vi "VIH Utility - FILE - Save File Dialog.vi"(4 "pattern label":string, 5 "button label":string, 6 "pattern":string, 7 "prompt":string, 8 "error in":errorcluster, 9 "default name":string, 11 "start path":path) -> (0 "error out":errorcluster, 2 "exists":bool, 3 "File path":path)   [LabVIEW 2014]
doc: "::: VI Helpeks :::\nCopyright (c) 2000-2026 Konstantin Shifershteyn. All rights reserved."
panel:
  # "VI Helpeks\nCopyright (c) 2012-2026 Konstantin Shifershteyn"
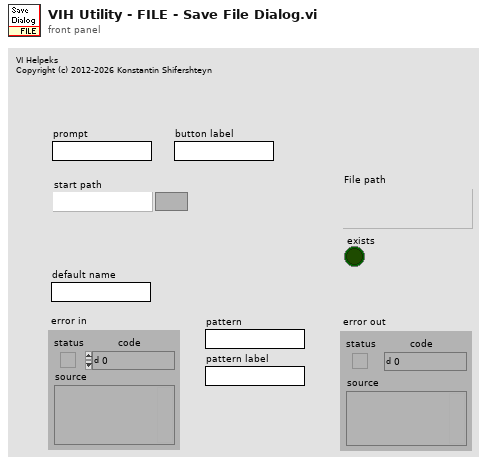
[diagram p1: front panel]
types:
  T1 = cluster{"Left Button Key Shortcut":cluster{"Control":bool, "Shift":bool, "Key":string}, "Center Button Key Shortcut":cluster{"Control":bool, "Shift":bool, "Key":string}, "Right Button Key Shortcut":cluster{"Control":bool, "Shift":bool, "Key":string}}
  T2 = enum16{"Left Button", "Center Button", "Right Button", "Window Close"}
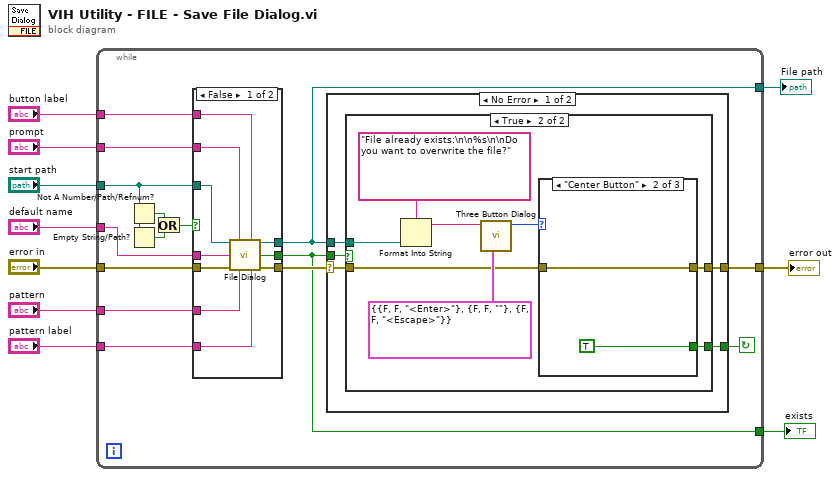
[diagram p0: block diagram]
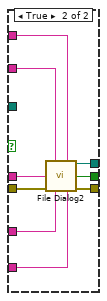
[diagram p2: hidden frame]
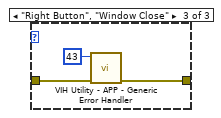
[diagram p5: hidden frame]
diagram:
  n1 = while {
    tunnel: [w22] -> w10
    tunnel: [w24] -> w9
    tunnel: [w21] -> w8
    tunnel: "error in" -> [w20]
    tunnel: "pattern" -> [w19]
    tunnel: "pattern label" -> [w18]
    tunnel: "default name" -> [w17]
    tunnel: "start path" -> [w12]
    tunnel: "prompt" -> [w16]
    tunnel: "button label" -> [w15]
    stop <- w25 continue-if-true
    n2 = Not A Number/Path/Refnum?(number/path/refnum=w12) -> (NaN/Path/Refnum?=w14:bool)
    n3 = Empty String/Path?(string/path=w12) -> (empty?=w13:bool)
    n4 = Or(x=w14, y=w13) -> (x .or. y?=w11:bool)
    n5 = case shown="False" w11 {
      tunnel: [w35 w44] -> w23
      tunnel: [w34 w43] -> w22
      tunnel: [w33 w42] -> w21
      tunnel: w20 -> [w32 w41]
      tunnel: w19 -> [w31 w40]
      tunnel: w18 -> [w30 w39]
      tunnel: w17 -> [w29 w38]
      tunnel: w12 -> [w28 _]
      tunnel: w16 -> [w27 w37]
      tunnel: w15 -> [w26 w36]
      frame False {
        n6 = call "File Dialog"("start path"=w28, "prompt"=w27, "button label"=w26, "default name"=w29, "error in"=w32, "pattern (all files)"=w31, "pattern label"=w30) -> ("selected path"=w34:path, "exists"=w33:bool, "error out"=w35:errorcluster)  [unwired: 5 in, 1 out]
      }
      frame True {
        n7 = call "File Dialog2"("prompt"=w37, "button label"=w36, "default name"=w38, "error in"=w41, "pattern (all files)"=w40, "pattern label"=w39) -> ("selected path"=w43:path, "exists"=w42:bool, "error out"=w44:errorcluster)  [unwired: 6 in, 1 out]
      }
    }
    n8 = case shown="No Error" w23 {
      selector: w23 -> [w46 w65]
      tunnel: w22 -> [w48 _]
      tunnel: w21 -> [w49 _]
      tunnel: [w47 _] -> w25
      tunnel: [w45 w65] -> w24
      frame No Error {
        n9 = case shown="True" w49 {
          tunnel: w48 -> [_ w58]
          tunnel: [_ w53] -> w47
          tunnel: w46 -> [w50 w51]
          tunnel: [w50 w52] -> w45
          frame False {
          }
          frame True {
            n10 = Format Into String(format string="File already exists:\n\n%s\n\nDo you want to overwrite the file?", w58) -> (resulting string=w56:string)  [unwired: 2 in, 1 out]
            n11 = call <vilib>:"Three Button Dialog.vi"("Keyboard Shortcuts (Left is <Enter>)"=T1 {"Left Button Key Shortcut"={"Control"=FALSE, "Shift"=FALSE, "Key"="<Enter>"}, "Center Button Key Shortcut"={"Control"=FALSE, "Shift"=FALSE, "Key"=""}, "Right Button Key Shortcut"={"Control"=FALSE, "Shift"=FALSE, "Key"="<Escape>"}}, "message"=w56) -> ("Which Button?"=w54:T2)  [unwired: 4 in, 5 out]
            n12 = case shown="\"Center Button\"" w54 {
              tunnel: [_ TRUE _] -> w53
              tunnel: [w59 w60 w64] -> w52
              tunnel: w51 -> [w59 w60 w63]
              frame "Left Button" {
              }
              frame "Center Button" {
              }
              frame "Right Button", "Window Close" {
                n13 = call "VIH Utility - APP - Generic Error Handler.vi"("error in"=w63, "error code"=43) -> ("error out"=w64:errorcluster)  [unwired: 9 out]
              }
            }
          }
        }
      }
      frame Error {
      }
    }
  }
  "File path" <- w10
  "error out" <- w9
  "exists" <- w8
